vi "thermal_optical_capture_19.vi"() -> ()   [LabVIEW 2025]
uses:
  <vilib>/vision/driver/IMAQdx.llb/IMAQdx Acquisition Mode.ctl
  <vilib>/vision/driver/IMAQdx.llb/IMAQdx Buffer Number Mode.ctl
  <vilib>/vision/driver/NI_Vision_Acquisition_Software.lvlib
panel:
  out "Optical Preview":T1(plugin-control)
  out "Optical Frame Out":string
  out "FPS":u32
  in  "Camera Name":refnum<k21> caption="IMAQdx Session"
  in  "milliseconds to wait":u32=100
  out "Thermal Preview":T1(plugin-control)
  in  "Stop Preview":bool
  in  "STOP ACQUISITION":bool
  in  "Focus":dbl(slide) scale=0.0..100.0
  out "Thermal Frame Out":string
  in  "Output Folder":path
  in  "thermal capture interval (s)":dbl
  in  "Flag Button":bool
  in  "Stop & Save":bool
  in  "Record":bool
  # "Instructions:\n1) Make sure terminal is closed (from previous sessions)\n2) Inputs: Select camera, data folder path, & milliseconds to wait (~100)\n3) Run VI. (Optical images will begin writing, disregard.)\n4) Wait until terminal gives \"thermal camera calibrated and data reliable\" message\n5) Press Thermal Record \"Start\", both thermal & optical will write files with common timestamps"
  # "Thermal Record"
  # "(Enter \"28\")"
  # "^ append to base data folder \"...\\raw\\test_n\" for nth recording"
  # "(applies to thermal)"
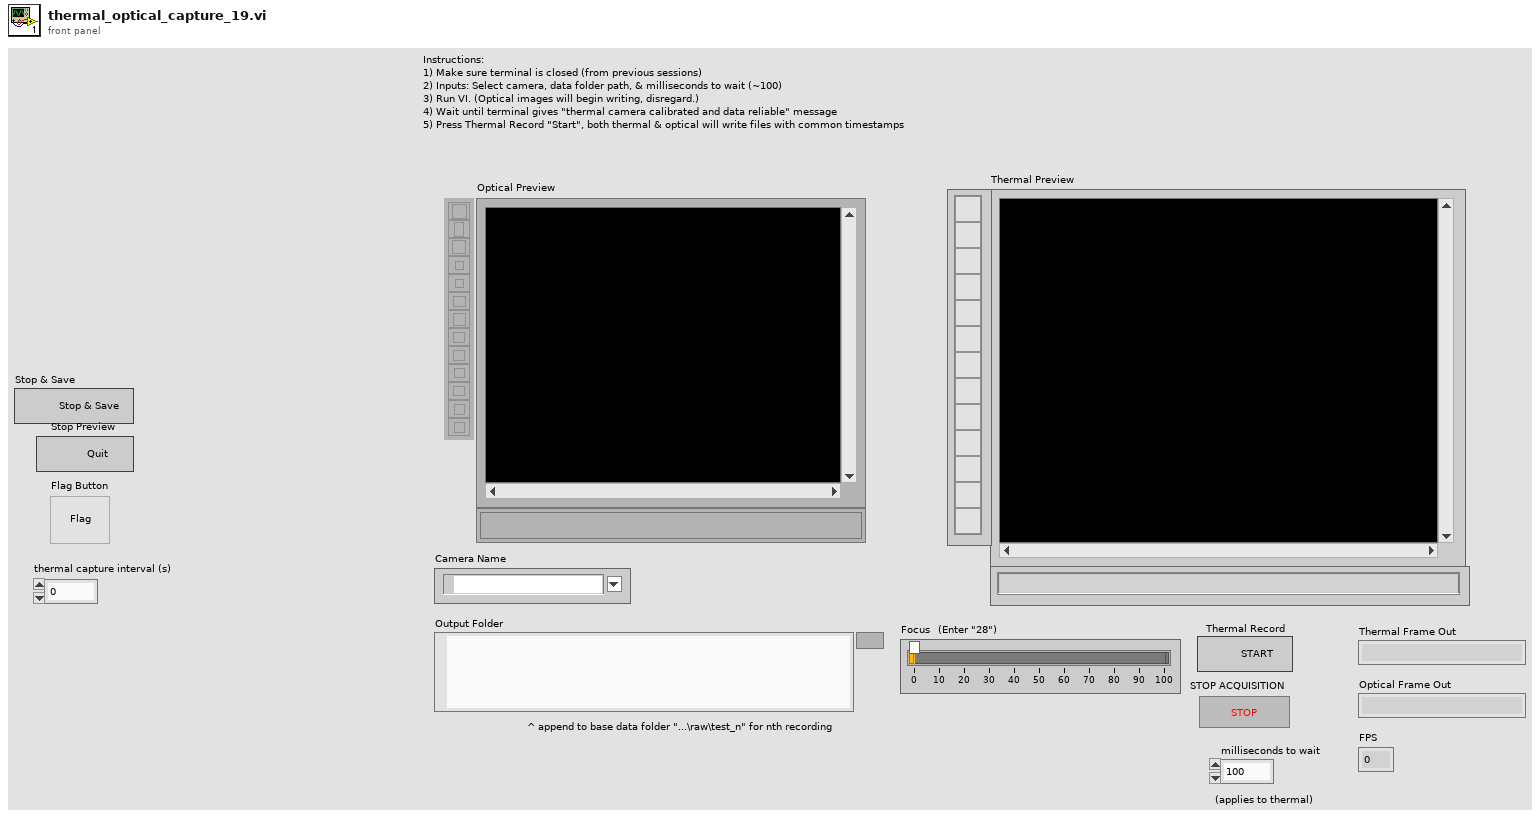
[diagram p1: front panel]
types:
  T1 = typedef "IMAQ Image.ctl" = refnum<image>
  T2 = typedef "NI_Vision_Acquisition_Software.lvlib/IMAQdx Acquisition Mode.ctl" = enum32{"One Shot", "Continuous"}
  T3 = enum16{"open", "replace", "create", "open or create", "replace or create", "replace or create with confirmation"}
  T4 = enum16{"big-endian, network order", "native, host order", "little-endian"}
  T5 = typedef "NI_Vision_Acquisition_Software.lvlib/IMAQdx Buffer Number Mode.ctl" = enum32{"Next", "Last", "Buffer Number", "Every", "Last New"}
  T6 = typedef "Image Type" = u32
  T7 = typedef "IMAQdx.ctl" = refnum<k21>
  T8 = enum16{"Standard", "Buffered", "CRLF", "Immediate"}
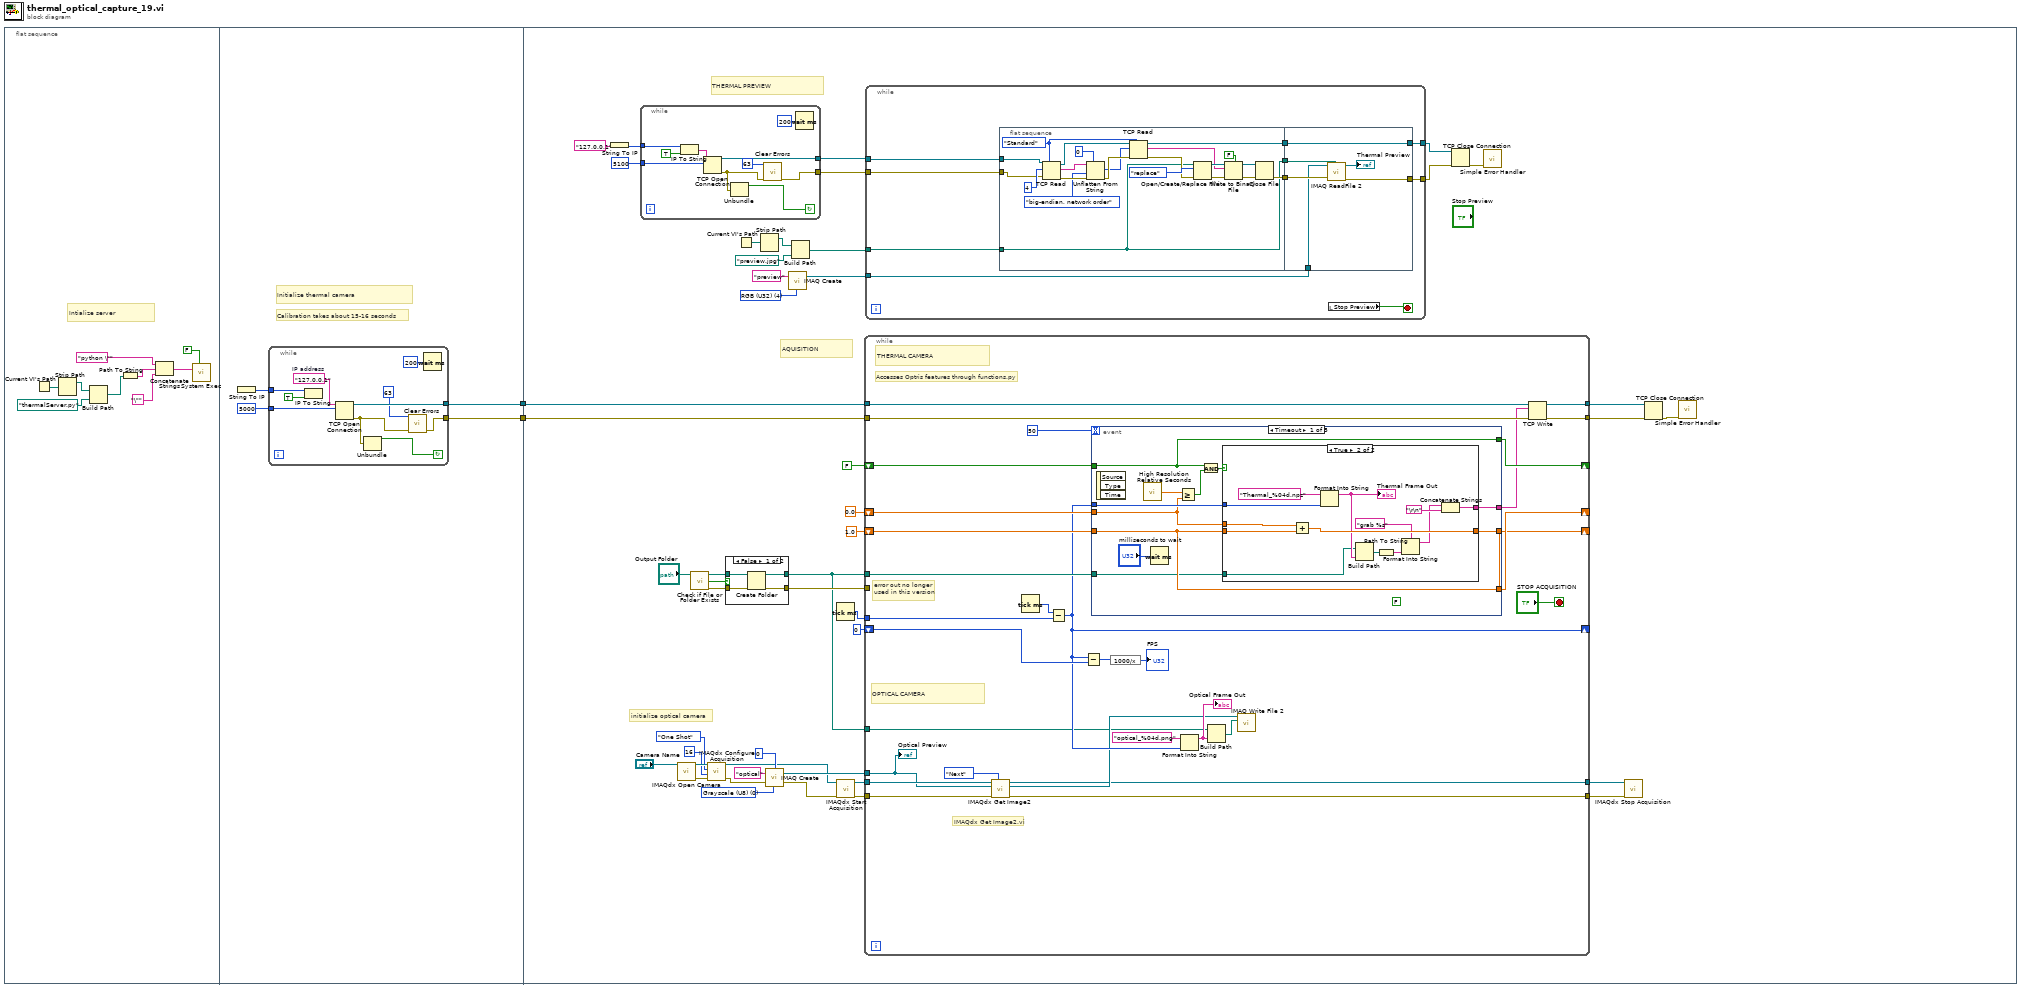
[diagram p0: block diagram]
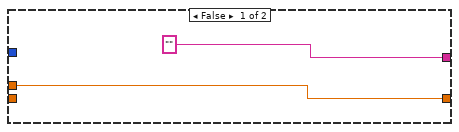
[diagram p3: hidden frame]
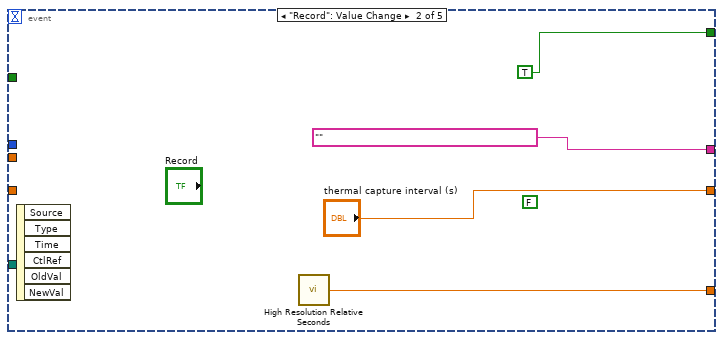
[diagram p4: hidden frame]
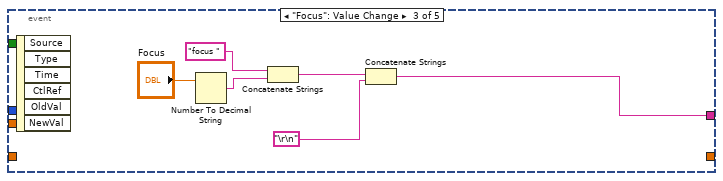
[diagram p5: hidden frame]
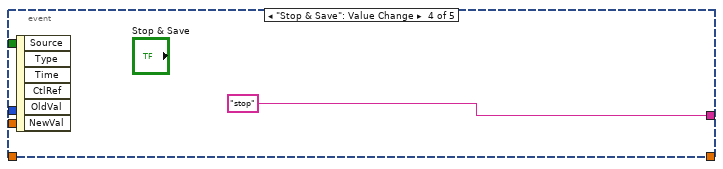
[diagram p6: hidden frame]
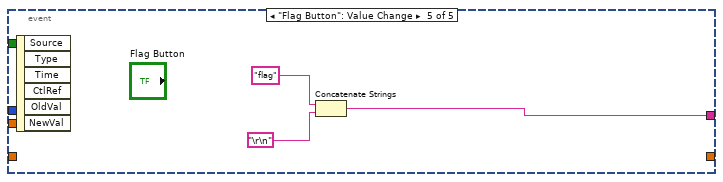
[diagram p7: hidden frame]
diagram:
  n1 = flat-sequence {
    tunnel: [w13] -> w2
    tunnel: [w12] -> w1
    tunnel: w1 -> [w68]
    tunnel: w2 -> [w67]
    frame #0 {
      # "Intialize server"
      n2 = Current VI's Path() -> (path=w6:path)
      n3 = Strip Path(path=w6) -> (stripped path=w7:path)  [unwired: 1 out]
      n4 = Build Path(base path=w7, name or relative path=path "thermalServer.py") -> (appended path=w4:path)
      n5 = Path To String(path=w4) -> (string=w10:string)
      n6 = Concatenate Strings("python \"" ("string"), w10, "\"" ("string")) -> (w9:string)
      n7 = call <vilib>:"System Exec.vi"("wait until completion? (T)"=FALSE, "command line"=w9) -> ()  [unwired: 6 in, 4 out]
    }
    frame #1 {
      # "Initialize thermal camera"
      # "Calibration takes about 15-16 seconds"
      n8 = String To IP() -> (0:w15:u32)  [unwired: 1 in]
      n9 = while {
        tunnel: [w20] -> w13
        tunnel: [w25] -> w12
        tunnel: w15 -> [w24]
        tunnel: u16 5000 ("remote port or service name") -> [w22]
        stop <- w17 continue-if-true
        w16 = "127.0.0.1"  # IP address
        n10 = IP To String(1:TRUE ("dot notation? (F)"), 2:w24) -> ()  [unwired: 1 out]
        n11 = TCP Open Connection(address=w16, remote port or service name=w22) -> (connection ID=w25:refnum<k5>, error out=w21:errorcluster)  [unwired: 3 in]
        n12 = Unbundle(w21) -> ("status"=w17:bool)  [unwired: 2 out]
        n13 = call <vilib>:"Clear Errors.vi"("error in (no error)"=w21, "specific error code to clear (0: all)"=63) -> ("error out"=w20:errorcluster)  [unwired: 4 in, 1 out]
        n14 = Wait (ms)(milliseconds to wait=u32 200) -> ()  [unwired: 1 out]
      }
    }
    frame #2 {
      w36 = T6 0 items=["Grayscale (U8)", "Grayscale (I16)", "Grayscale (SGL)", "Complex (CSG)", "RGB (U32)", "HSL (U32)", "RGB (U64)", "Grayscale (U16)"] ("Image Type")
      w56 = T6 4 items=["Grayscale (U8)", "Grayscale (I16)", "Grayscale (SGL)", "Complex (CSG)", "RGB (U32)", "HSL (U32)", "RGB (U64)", "Grayscale (U16)"] ("Image Type")
      # "initialize optical camera"
      # "THERMAL PREVIEW"
      # "AQUISITION"
      n15 = String To IP(1:"127.0.0.1" ("name")) -> (0:w55:u32)
      n16 = while {
        tunnel: w55 -> [w87]
        tunnel: [w81] -> w54
        tunnel: [w85] -> w53
        tunnel: u16 5100 ("remote port or service name") -> [w83]
        stop <- w78 continue-if-true
        n17 = IP To String(1:TRUE ("dot notation? (F)"), 2:w87) -> (0:w86:string)
        n18 = TCP Open Connection(address=w86, remote port or service name=w83) -> (connection ID=w85:refnum<k5>, error out=w82:errorcluster)  [unwired: 3 in]
        n19 = Unbundle(w82) -> ("status"=w78:bool)  [unwired: 2 out]
        n20 = call <vilib>:"Clear Errors.vi"("error in (no error)"=w82, "specific error code to clear (0: all)"=63) -> ("error out"=w81:errorcluster)  [unwired: 4 in, 1 out]
        n21 = Wait (ms)(milliseconds to wait=u32 200) -> ()  [unwired: 1 out]
      }
      n22 = call <vilib>:"IMAQdx Open Camera.vi"("Session In"="Camera Name") -> ("error out"=w41:errorcluster, "Session Out"=w42:T7)  [unwired: 9 in]
      n23 = call <vilib>:"Check if File or Folder Exists.vi"("path"="Output Folder") -> ("error out"=w48:errorcluster, "file or folder exists?"=w50:bool)  [unwired: 8 in, 1 out]
      n24 = call <vilib>:"IMAQdx Configure Acquisition.vi"("error in"=w41, "Number of Buffers"=u32 16, "Continuous?"=IMAQdx_Acquisition_Mode."One Shot", "Session In"=w42) -> ("error out"=w39:errorcluster, "Session Out"=w32:T7)  [unwired: 6 in]
      n25 = case shown="False" w50 {
        tunnel: "Output Folder" -> [w75 w77]
        tunnel: [w74 w77] -> w31
        tunnel: w48 -> [w73 w76]
        tunnel: [w72 w76] -> w47
        frame False {
          n26 = Create Folder(path (use dialog)=w75, error in=w73) -> (created path=w74:path, error out=w72:errorcluster)  [unwired: 1 in, 1 out]
        }
        frame True {
        }
      }
      n27 = Current VI's Path() -> (path=w61:path)
      n28 = Strip Path(path=w61) -> (stripped path=w62:path)  [unwired: 1 out]
      n29 = call "IMAQ Create"("Border Size"=0, "Image Name"="optical", "Image Type"=w36, "error in (no error)"=w39) -> ("New Image"=w33:T1, "error out"=w28:errorcluster)  [unwired: 1 in]
      n30 = call "IMAQ Create"("Image Name"="preview", "Image Type"=w56) -> ("New Image"=w59:T1)  [unwired: 3 in, 1 out]
      n31 = Build Path(base path=w62, name or relative path=path "preview.jpg") -> (appended path=w60:path)
      n32 = Tick Count (ms)() -> (millisecond timer value=w63:u32)
      n33 = call <vilib>:"IMAQdx Start Acquisition.vi"("error in"=w28, "Session In"=w32) -> ("error out"=w27:errorcluster, "Session Out"=w26:T7)  [unwired: 8 in]
      n34 = while {
        tunnel: [w156] -> w69
        tunnel: [w155] -> w70
        tunnel: w68 -> [w154]
        tunnel: w67 -> [w153]
        shift-right: [w152] -> _
        shift-left: 0.0 -> [w149]
        shift-right: [w150] -> _
        shift-left: 1.0 -> [w147]
        shift-right: [w151] -> _
        shift-left: FALSE -> [w148]
        tunnel: w63 -> [w140]
        shift-right: [w139] -> _
        shift-left: u32 0 -> [w141]
        tunnel: w31 -> [w142]
        tunnel: w47 -> [_]
        tunnel: w33 -> [w128]
        tunnel: w31 -> [w133]
        tunnel: [w135] -> w30
        tunnel: [w134] -> w29
        tunnel: w27 -> [w130]
        tunnel: w26 -> [w129]
        stop <- "STOP ACQUISITION" stop-if-true
        # "IMAQdx Get Image2.vi"
        # "OPTICAL CAMERA"
        # "error out no longer used in this version"
        # "THERMAL CAMERA"
        # "Accesses Optris features through functions.py"
        n35 = call <vilib>:"IMAQdx Get Image2.vi"("Buffer Number Mode (Next)"=IMAQdx_Buffer_Number_Mode."Next", "error in"=w130, "Image In"=w128, "Session In"=w129) -> ("error out"=w135:errorcluster, "Image Out"=w136:T1, "Session Out"=w134:T7)  [unwired: 4 in, 1 out]
        n36 = Tick Count (ms)() -> (millisecond timer value=w143:u32)
        n37 = Subtract(x=w143, y=w140) -> (x-y=w139:u32)
        n38 = Subtract(x=w139, y=w141) -> (x-y=w127:u32)
        n39 = event shown="[0] Timeout" {
          selector: _ -> [_ _ _ _ _]
          dyn-events: _ -> [_ _ _ _ _]
          timeout: 50 -> [_ _ _ _ _]
          tunnel: [w163 "" w187 "stop" w196] -> w144
          tunnel: w139 -> [w164 _ _ _ _]
          tunnel: [w161 w186 _ _ _] -> w152
          tunnel: [w159 TRUE _ _ _] -> w151
          tunnel: [w160 "thermal capture interval (s)" _ _ _] -> w150
          tunnel: w149 -> [w162 _ _ _ _]
          tunnel: w148 -> [w159 _ _ _ _]
          tunnel: w147 -> [w160 _ _ _ _]
          tunnel: w142 -> [w158 _ _ _ _]
          event Timeout {
            (unwired) FALSE
            n40 = event-data() -> ()  [unwired: 1 in, 3 out]
            n41 = call <vilib>:"High Resolution Relative Seconds.vi"() -> ("relative seconds"=w167:dbl)
            n42 = Wait (ms)(milliseconds to wait="milliseconds to wait") -> ()  [unwired: 1 out]
            n43 = Greater Or Equal?(x=w167, y=w162) -> (x >= y?=w166:bool)
            n44 = And(x=w159, y=w166) -> (x .and. y?=w165:bool)
            n45 = case shown="True" w165 {
              tunnel: w164 -> [_ w180]
              tunnel: ["" w181] -> w163
              tunnel: w162 -> [w168 w179]
              tunnel: w160 -> [_ w178]
              tunnel: [w168 w177] -> w161
              tunnel: w158 -> [_ w170]
              frame False {
              }
              frame True {
                n46 = Add(x=w179, y=w178) -> (x+y=w177:dbl)
                n47 = Format Into String(format string="Thermal_%04d.npz", w180) -> (resulting string=w171:string)  [unwired: 2 in, 1 out]
                "Thermal Frame Out" <- w171
                n48 = Build Path(base path=w170, name or relative path=w171) -> (appended path=w175:path)
                n49 = Path To String(path=w175) -> (string=w173:string)
                n50 = Format Into String(format string="grab %s", w173) -> (resulting string=w172:string)  [unwired: 2 in, 1 out]
                n51 = Concatenate Strings(w172, "\r\n") -> (w181:string)
              }
            }
          }
          event "Record": Value Change {
            (unwired) FALSE
            n52 = event-data() -> ()  [unwired: 1 in, 6 out]
            n53 = call <vilib>:"High Resolution Relative Seconds.vi"() -> ("relative seconds"=w186:dbl)
          }
          event "Focus": Value Change {
            n54 = event-data() -> ()  [unwired: 1 in, 6 out]
            n55 = Number To Decimal String(number="Focus") -> (decimal integer string=w192:string)  [unwired: 1 in]
            n56 = Concatenate Strings("focus ", w192) -> (w189:string)
            n57 = Concatenate Strings(w189, "\r\n") -> (w187:string)
          }
          event "Stop & Save": Value Change {
            n58 = event-data() -> ()  [unwired: 1 in, 6 out]
          }
          event "Flag Button": Value Change {
            n59 = event-data() -> ()  [unwired: 1 in, 6 out]
            n60 = Concatenate Strings("flag", "\r\n") -> (w196:string)
          }
        }
        n61 = expression code="1000/x"(w127) -> (→"FPS":u32)
        n62 = Format Into String(format string="optical_%04d.png", w139) -> (resulting string=w137:string)  [unwired: 2 in, 1 out]
        "Optical Frame Out" <- w137
        n63 = Build Path(base path=w133, name or relative path=w137) -> (appended path=w131:path)
        n64 = call-poly "IMAQ Write File 2"("File Path"=w131, "Image"=w136) -> ()  [unwired: 8 in, 2 out]
        n65 = TCP Write(connection ID=w154, data in=w144, error in (no error)=w153) -> (connection ID out=w155:refnum<k5>, error out=w156:errorcluster)  [unwired: 1 in, 1 out]
        "Optical Preview" <- w128
      }
      n66 = while {
        tunnel: w59 -> [w92]
        tunnel: [w93] -> w45
        tunnel: [w97] -> w44
        tunnel: w60 -> [w95]
        tunnel: w54 -> [w90]
        tunnel: w53 -> [w89]
        stop <- w88 stop-if-true
        n67 = flat-sequence {
          tunnel: w95 -> [w101]
          tunnel: [w103] -> w96
          tunnel: [w102] -> w94
          tunnel: [w101] -> w91
          tunnel: w90 -> [w99]
          tunnel: w89 -> [w98]
          tunnel: [w125] -> w97
          tunnel: w96 -> [w125]
          tunnel: w94 -> [w124]
          tunnel: [w123] -> w93
          tunnel: w92 -> [w122]
          tunnel: w91 -> [w121]
          frame #0 {
            w112 = T8."Standard" ("mode (standard)")
            n68 = TCP Read(connection ID=w98, bytes to read=4, error in (no error)=w99, 7:w112) -> (connection ID out=w115:refnum<k5>, data out=w100:string, error out=w118:errorcluster)  [unwired: 1 in]
            n69 = Unflatten From String(type=0, binary string=w100, byte order (0:big-endian, network order)=T4."big-endian, network order", error in (no error)=w118) -> (value=w113:i32, error out=w114:errorcluster)  [unwired: 1 in, 1 out]
            n70 = TCP Read(connection ID=w115, bytes to read=w113, error in (no error)=w114, 7:w112) -> (connection ID out=w103:refnum<k5>, data out=w108:string, error out=w110:errorcluster)  [unwired: 1 in]
            n71 = Open/Create/Replace File(file path (use dialog)=w101, error in=w110, operation (0:open)=T3."replace") -> (refnum out=w109:refnum<file>, error out=w106:errorcluster)  [unwired: 3 in, 1 out]
            n72 = Write to Binary File(file (use dialog)=w109, data=w108, error in=w106, 5:FALSE ("prepend array or string size? (T)")) -> (refnum out=w104:refnum<file>, error out=w105:errorcluster)  [unwired: 2 in, 1 out]
            n73 = Close File(refnum=w104, error in=w105) -> (error out=w102:errorcluster)  [unwired: 1 out]
          }
          frame #1 {
            n74 = call "IMAQ ReadFile 2"("File Path"=w121, "error in (no error)"=w124, "Image"=w122) -> ("error out"=w123:errorcluster, "Image Out"=→"Thermal Preview":T1)  [unwired: 4 in, 3 out]
          }
        }
        n75 = local read "Stop Preview"() -> (w88:bool)
      }
      n76 = TCP Close Connection(connection ID=w44, error in (no error)=w45) -> (error out=w46:errorcluster)  [unwired: 1 in, 1 out]
      n77 = call <vilib>:"Simple Error Handler.vi"("error in (no error)"=w46) -> ()  [unwired: 4 in, 5 out]
      n78 = call <vilib>:"IMAQdx Stop Acquisition.vi"("error in"=w30, "Session In"=w29) -> ()  [unwired: 8 in, 2 out]
      n79 = TCP Close Connection(connection ID=w70, error in (no error)=w69) -> (error out=w71:errorcluster)  [unwired: 1 in, 1 out]
      n80 = call <vilib>:"Simple Error Handler.vi"("error in (no error)"=w71) -> ()  [unwired: 4 in, 5 out]
    }
  }
